vi "Read Scalar Data.vi"(8 "error in (no error)":errorcluster, 10 "Values":dbl[](array[numeric]), 11 "Cluster":T1 {"Data Type" format="%.0x"}) -> (0 "error out":errorcluster, 2 "Values":dbl[](array[numeric]), 3 "Cluster":T1 {"Data Type" format="%.0x"})   [LabVIEW 2019, in "FPGA Addon Engine.lvlib"]
uses:
  FPGA Addon Engine.lvlib
  Types/Register Settings.ctl
  Addon Shared/Types/Data Type.ctl
  Addon Shared/Types/Scalar Type.ctl
  <vilib>/Utility/error.llb/Error Cluster From Error Code.vi
  <vilib>/rvi/errors/niLvFpgaAdjustHostInterfaceError.vi
  <vilib>/rvi/interface/nirviReadWriteControl/nirviReadWriteControl.xnode
  NiFpgaLv.dll
  <vilib>/rvi/interface/Simulation/niFpgaSimulationCallBeginRW.vi
  Addon Shared/FPGA Addon Shared.lvlib
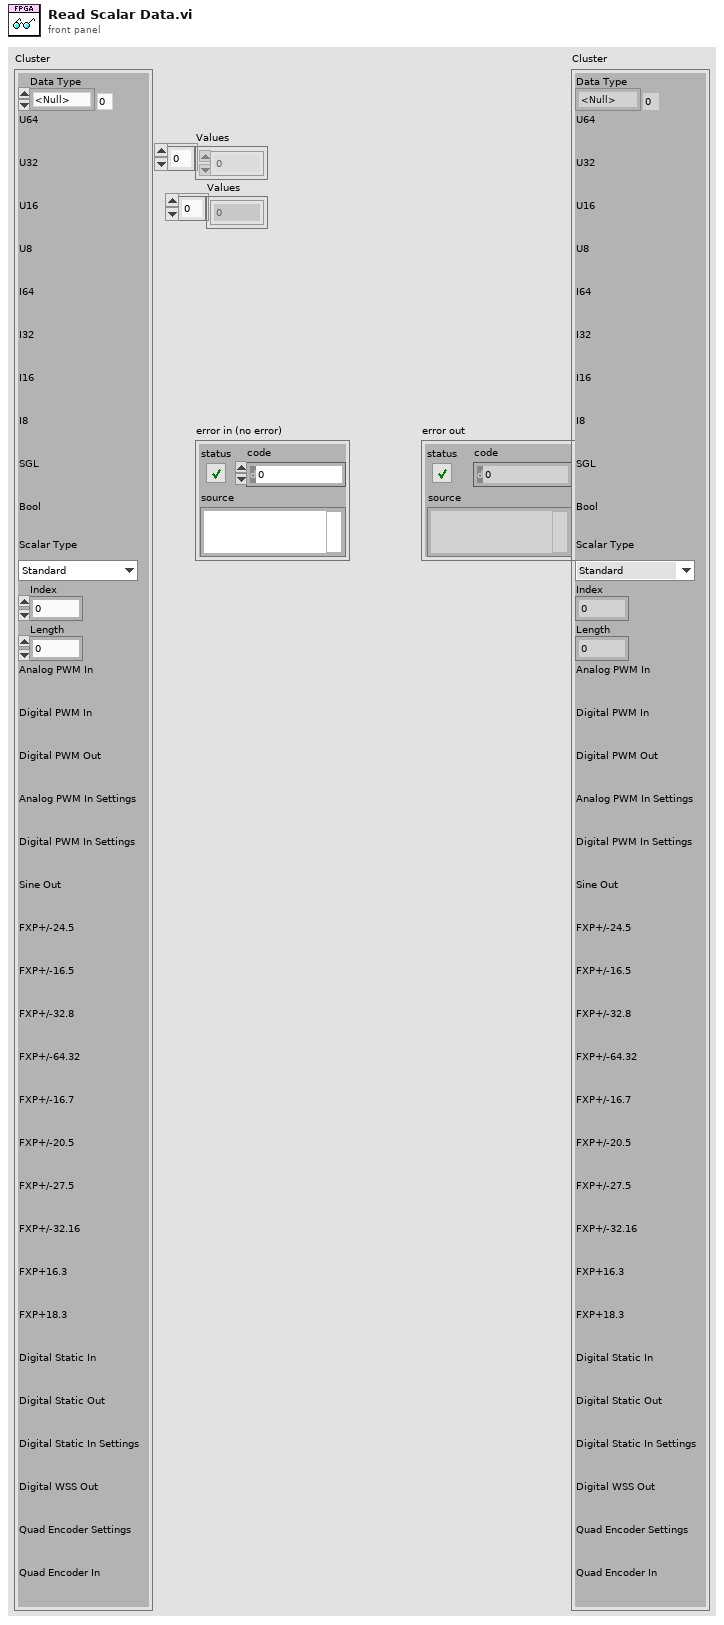
[diagram p1: front panel]
types:
  T1 = typedef "FPGA Addon Engine.lvlib/Register Settings.ctl" = cluster{"Data Type":T2, "U64":refnum<k20>, "U32":refnum<k20>, "U16":refnum<k20>, "U8":refnum<k20>, "I64":refnum<k20>, "I32":refnum<k20>, "I16":refnum<k20>, "I8":refnum<k20>, "SGL":refnum<k20>, "Bool":refnum<k20>, "Scalar Type":T3, "Index":i32, "Length":i32, "Analog PWM In":refnum<k20>, "Digital PWM In":refnum<k20>, "Digital PWM Out":refnum<k20>, "Analog PWM In Settings":refnum<k20>, "Digital PWM In Settings":refnum<k20>, "Sine Out":refnum<k20>, "FXP+/-24.5":refnum<k20>, "FXP+/-16.5":refnum<k20>, "FXP+/-32.8":refnum<k20>, "FXP+/-64.32":refnum<k20>, "FXP+/-16.7":refnum<k20>, "FXP+/-20.5":refnum<k20>, "FXP+/-27.5":refnum<k20>, "FXP+/-32.16":refnum<k20>, "FXP+16.3":refnum<k20>, "FXP+18.3":refnum<k20>, "Digital Static In":refnum<k20>, "Digital Static Out":refnum<k20>, "Digital Static In Settings":refnum<k20>, "Digital WSS Out":refnum<k20>, "Quad Encoder Settings":refnum<k20>, "Quad Encoder In":refnum<k20>}
  T2 = typedef "FPGA Addon Shared.lvlib/Data Type.ctl" = enum8{"<Null>", "I8", "I16", "I32", "I64", "U8", "U16", "U32", "U64", "SGL", "Boolean", "Analog PWM In Settings", "Analog PWM In", "Digital PWM In Settings", "Digital PWM In", "Digital PWM Out", "Sine Out", "FXP+/-24.5", "FXP+/-16.5", "FXP+/-32.8", "FXP+/-64.32", "FXP+/-16.7", "FXP+/-20.5", "FXP+/-27.5", "FXP+/-32.16", "FXP +16.3", "FXP +18.3", "Digital Static In", "Digital Static Out", "Digital Static In Settings", "Digital WSS Out", "Quad Encoder Settings", "Quad Encoder In"}
  T3 = typedef "FPGA Addon Shared.lvlib/Scalar Type.ctl" = enum16{"Standard", "Bitpacked"}
  T4 = cluster{"ACTIVE TICKS":u32, "INACTIVE TICKS":u32, "ACQ TICKS":u32, "ACTIVE VOLTAGE":fxp<+/-,32,8>, "INACTIVE VOLTAGE":fxp<+/-,32,8>}
  T5 = cluster{"ACTIVE TICKS":u32, "INACTIVE TICKS":u32, "ACQ TICKS":u32}
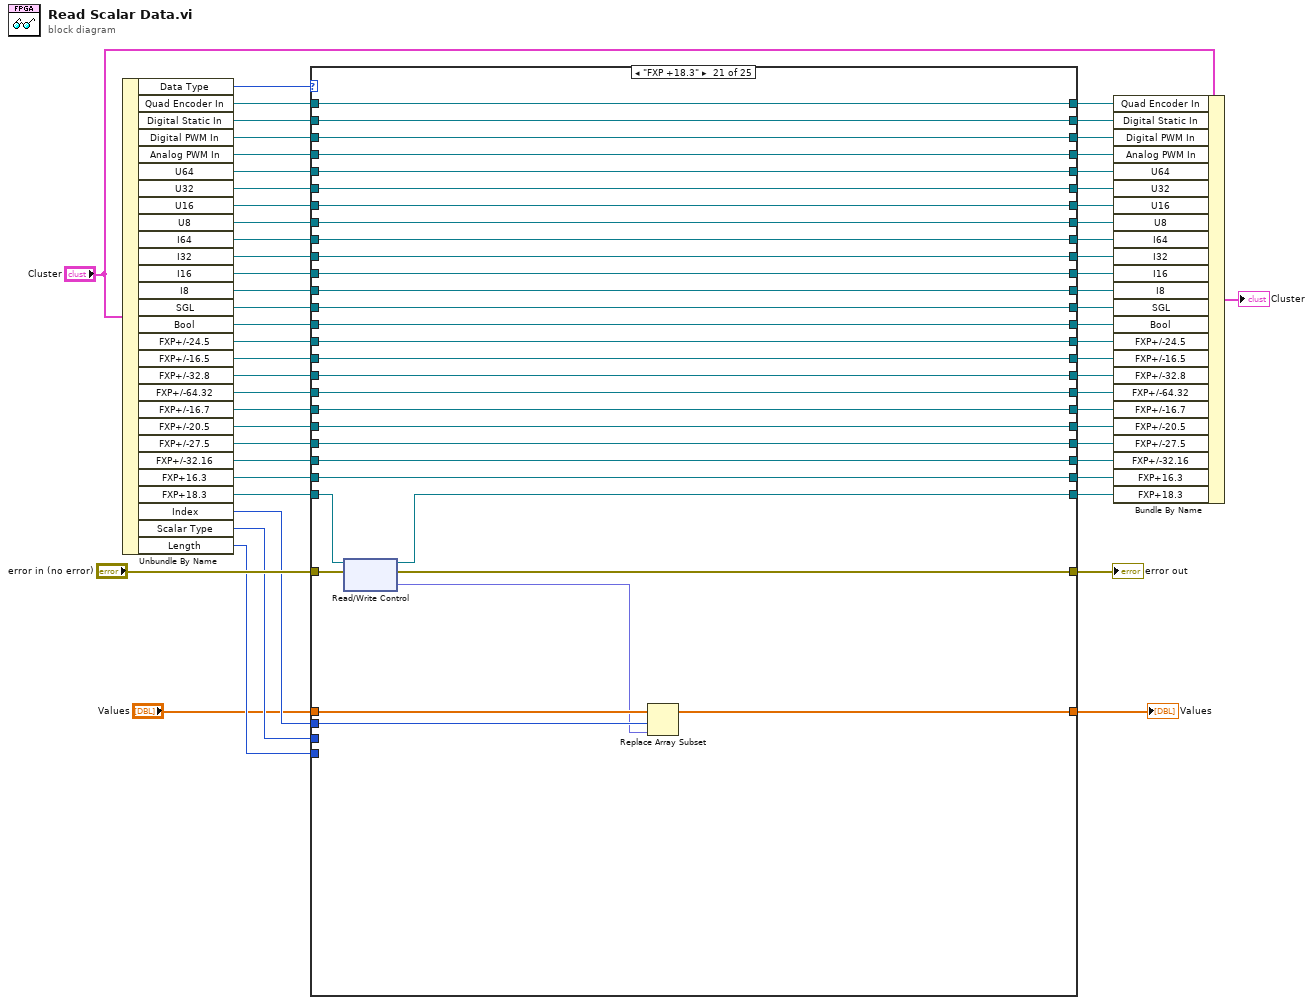
[diagram p0: block diagram]
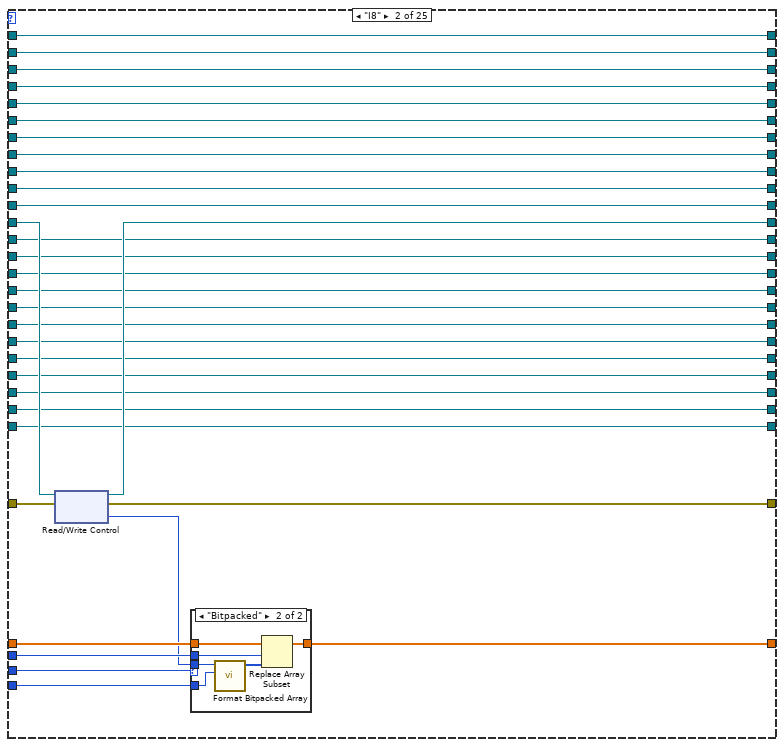
[diagram p3: hidden frame]
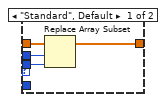
[diagram p4: hidden frame]
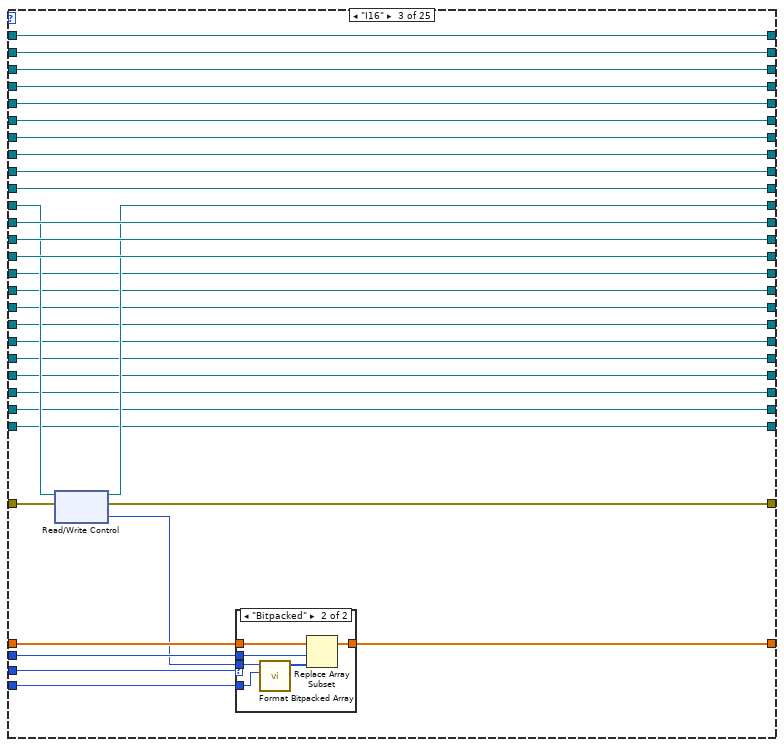
[diagram p5: hidden frame]
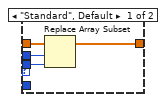
[diagram p6: hidden frame]
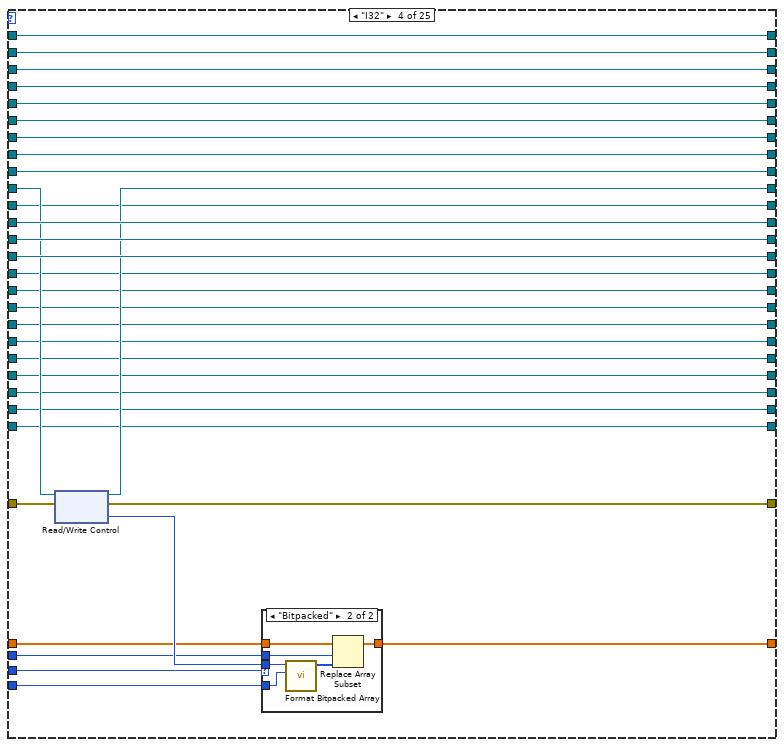
[diagram p7: hidden frame]
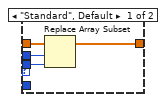
[diagram p8: hidden frame]
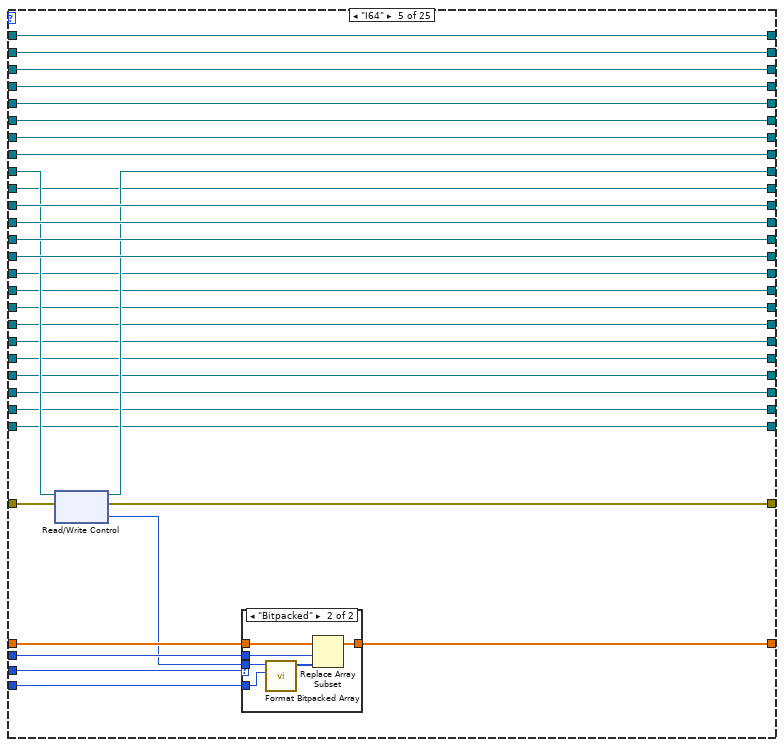
[diagram p9: hidden frame]
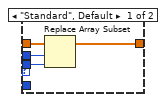
[diagram p10: hidden frame]
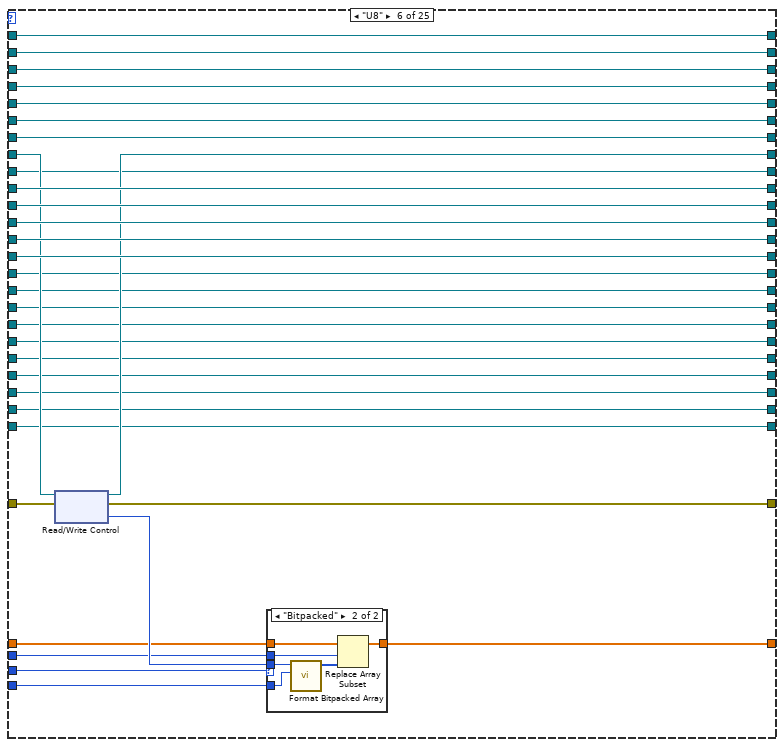
[diagram p11: hidden frame]
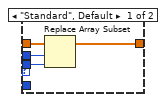
[diagram p12: hidden frame]
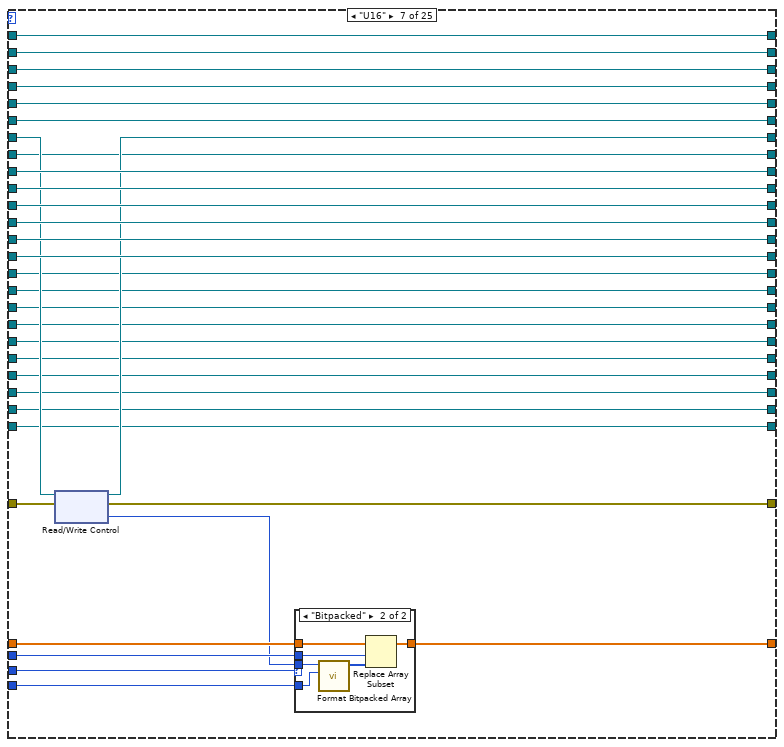
[diagram p13: hidden frame]
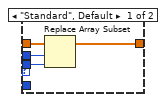
[diagram p14: hidden frame]
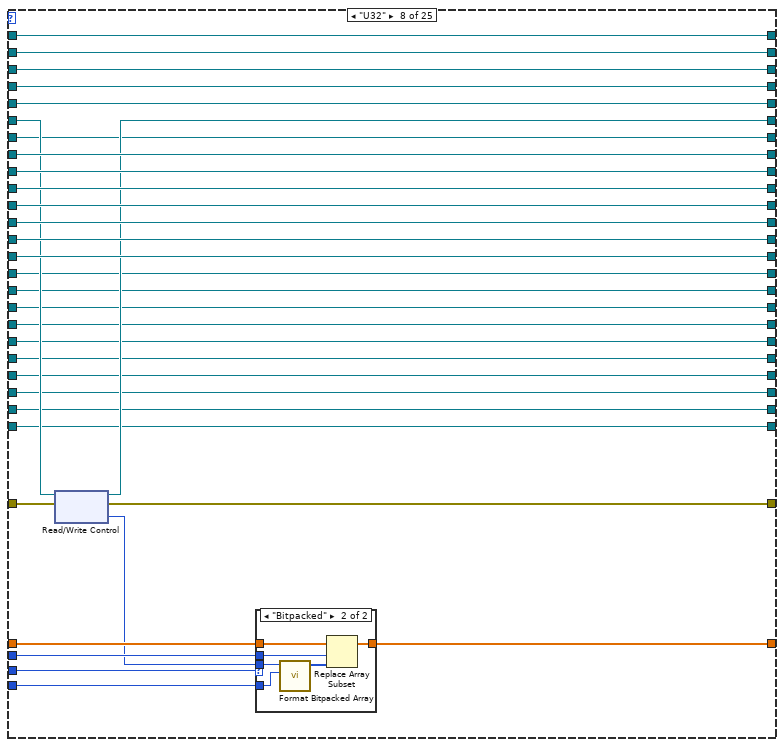
[diagram p15: hidden frame]
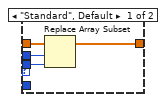
[diagram p16: hidden frame]
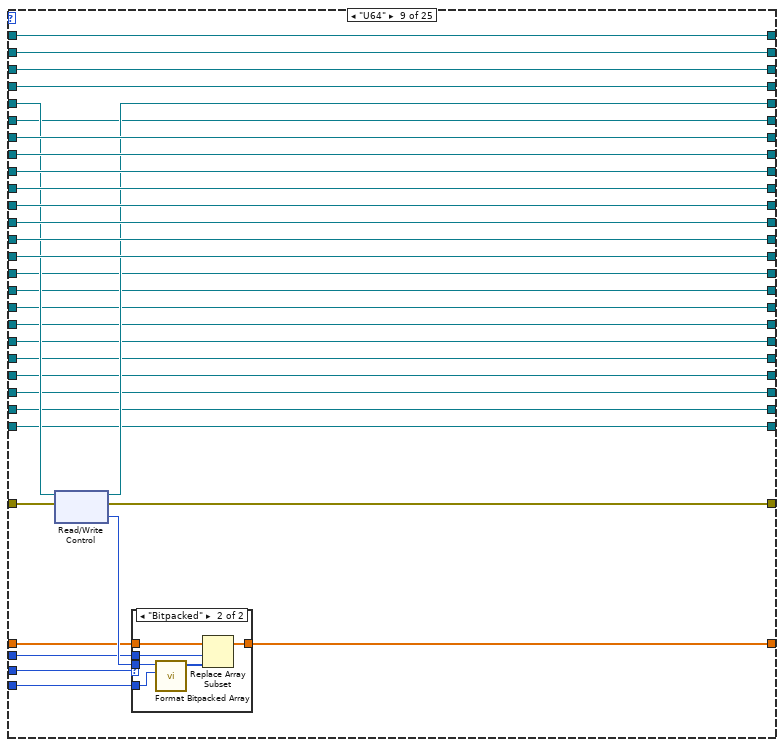
[diagram p17: hidden frame]
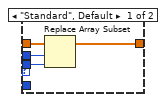
[diagram p18: hidden frame]
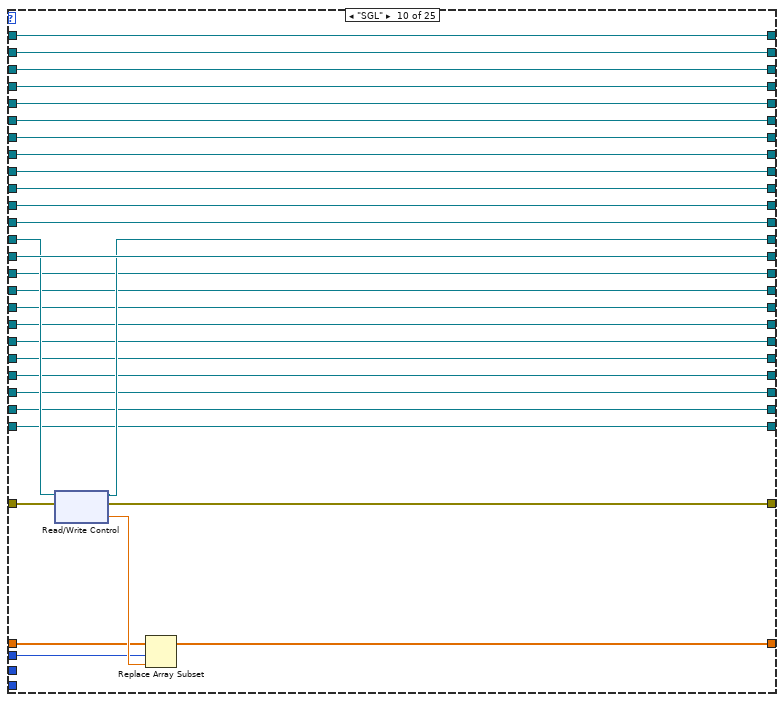
[diagram p19: hidden frame]
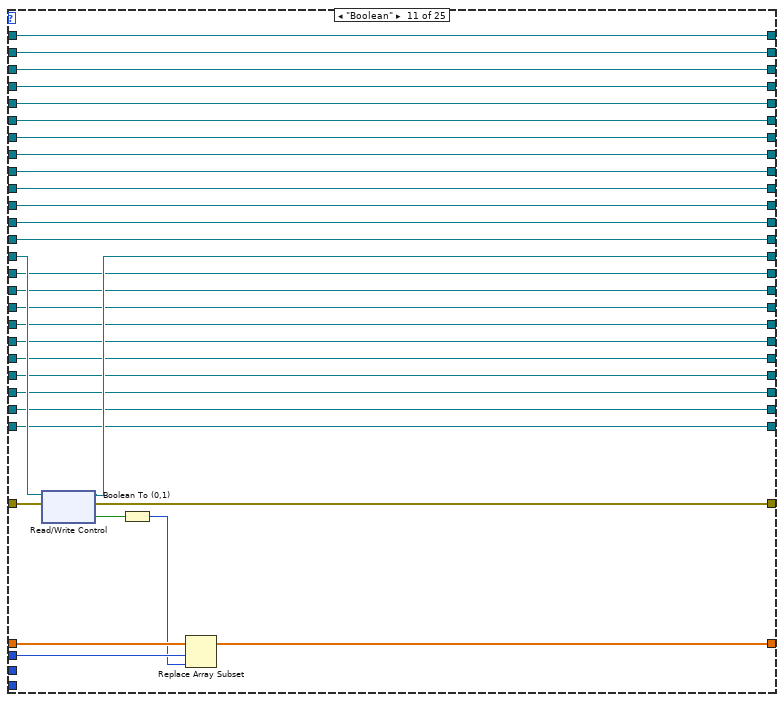
[diagram p20: hidden frame]
diagram:
  n1 = Unbundle By Name("Cluster") -> ("Data Type"=w7:T2, "Quad Encoder In"=w6:refnum<k20>, "Digital Static In"=w9:refnum<k20>, "Digital PWM In"=w27:refnum<k20>, "Analog PWM In"=w28:refnum<k20>, "U64"=w36:refnum<k20>, "U32"=w38:refnum<k20>, "U16"=w40:refnum<k20>, "U8"=w42:refnum<k20>, "I64"=w44:refnum<k20>, "I32"=w46:refnum<k20>, "I16"=w48:refnum<k20>, "I8"=w58:refnum<k20>, "SGL"=w52:refnum<k20>, "Bool"=w51:refnum<k20>, "FXP+/-24.5"=w25:refnum<k20>, "FXP+/-16.5"=w22:refnum<k20>, "FXP+/-32.8"=w21:refnum<k20>, "FXP+/-64.32"=w18:refnum<k20>, "FXP+/-16.7"=w16:refnum<k20>, "FXP+/-20.5"=w14:refnum<k20>, "FXP+/-27.5"=w13:refnum<k20>, "FXP+/-32.16"=w10:refnum<k20>, "FXP+16.3"=w3:refnum<k20>, "FXP+18.3"=w1:refnum<k20>, "Index"=w32:i32, "Scalar Type"=w33:T3, "Length"=w34:i32)
  n2 = case shown="\"FXP +18.3\"" w7 {
    tunnel: w58 -> [w82 w117 w150 w194 w238 w282 w326 w370 w414 w456 w489 w520 w551 w582 w613 w644 w675 w706 w737 w768 w799 w832 w878 w934 w971]
    tunnel: "error in (no error)" -> [w74 w116 w160 w203 w246 w289 w332 w375 w418 w459 w491 w522 w553 w584 w615 w646 w677 w708 w739 w770 w801 w834 w875 w931 w968]
    tunnel: [w74 w115 w159 w202 w245 w288 w331 w374 w417 w458 w490 w521 w552 w583 w614 w645 w676 w707 w738 w769 w800 w833 w874 w930 w967] -> w56
    tunnel: [w82 w114 w150 w194 w238 w282 w326 w370 w414 w456 w489 w520 w551 w582 w613 w644 w675 w706 w737 w768 w799 w832 w878 w934 w971] -> w54
    tunnel: [w83 w113 w158 w201 w244 w287 w330 w373 w416 w447 w479 w512 w543 w574 w605 w636 w667 w698 w729 w760 w791 w824 w877 w933 w970] -> w53
    tunnel: w52 -> [w83 w113 w158 w201 w244 w287 w330 w373 w416 w449 w479 w512 w543 w574 w605 w636 w667 w698 w729 w760 w791 w824 w877 w933 w970]
    tunnel: w51 -> [w84 w112 w157 w200 w243 w286 w329 w372 w415 w457 w481 w505 w537 w568 w599 w630 w661 w692 w723 w754 w785 w818 w876 w932 w969]
    tunnel: [w84 w112 w157 w200 w243 w286 w329 w372 w415 w457 w480 w505 w537 w568 w599 w630 w661 w692 w723 w754 w785 w818 w876 w932 w969] -> w50
    tunnel: [w81 w111 w148 w191 w237 w281 w325 w369 w413 w455 w488 w519 w550 w581 w612 w643 w674 w705 w736 w767 w798 w831 w879 w935 w972] -> w49
    tunnel: w48 -> [w81 w111 w149 w191 w237 w281 w325 w369 w413 w455 w488 w519 w550 w581 w612 w643 w674 w705 w736 w767 w798 w831 w879 w935 w972]
    tunnel: [w80 w110 w156 w192 w234 w280 w324 w368 w412 w454 w487 w518 w549 w580 w611 w642 w673 w704 w735 w766 w797 w830 w880 w936 w973] -> w47
    tunnel: w46 -> [w80 w110 w156 w193 w234 w280 w324 w368 w412 w454 w487 w518 w549 w580 w611 w642 w673 w704 w735 w766 w797 w830 w880 w936 w973]
    tunnel: [w79 w109 w155 w199 w235 w277 w323 w367 w411 w453 w486 w517 w548 w579 w610 w641 w672 w703 w734 w765 w796 w829 w881 w937 w974] -> w45
    tunnel: w44 -> [w79 w109 w155 w199 w236 w277 w323 w367 w411 w453 w486 w517 w548 w579 w610 w641 w672 w703 w734 w765 w796 w829 w881 w937 w974]
    tunnel: [w78 w108 w154 w198 w242 w278 w320 w366 w410 w452 w485 w516 w547 w578 w609 w640 w671 w702 w733 w764 w795 w828 w882 w938 w975] -> w43
    tunnel: w42 -> [w78 w108 w154 w198 w242 w279 w320 w366 w410 w452 w485 w516 w547 w578 w609 w640 w671 w702 w733 w764 w795 w828 w882 w938 w975]
    tunnel: [w77 w107 w153 w197 w241 w285 w321 w363 w409 w451 w484 w515 w546 w577 w608 w639 w670 w701 w732 w763 w794 w827 w883 w939 w976] -> w41
    tunnel: w40 -> [w77 w107 w153 w197 w241 w285 w322 w363 w409 w451 w484 w515 w546 w577 w608 w639 w670 w701 w732 w763 w794 w827 w883 w939 w976]
    tunnel: [w76 w106 w152 w196 w240 w284 w328 w364 w406 w450 w483 w514 w545 w576 w607 w638 w669 w700 w731 w762 w793 w826 w884 w940 w977] -> w39
    tunnel: w38 -> [w76 w106 w152 w196 w240 w284 w328 w365 w406 w450 w483 w514 w545 w576 w607 w638 w669 w700 w731 w762 w793 w826 w884 w940 w977]
    tunnel: [w75 w105 w151 w195 w239 w283 w327 w371 w407 w448 w482 w513 w544 w575 w606 w637 w668 w699 w730 w761 w792 w825 w885 w941 w978] -> w37
    tunnel: w36 -> [w75 w105 w151 w195 w239 w283 w327 w371 w408 w448 w482 w513 w544 w575 w606 w637 w668 w699 w730 w761 w792 w825 w885 w941 w978]
    tunnel: w34 -> [_ w101 w144 w185 w230 w273 w319 w358 w402 _ _ _ _ _ _ _ _ _ _ _ _ _ _ _ _]
    tunnel: w33 -> [_ w102 w145 w186 w231 w272 w318 w359 w403 _ _ _ _ _ _ _ _ _ _ _ _ _ _ _ _]
    tunnel: w32 -> [_ w103 w146 w189 w232 w274 w317 w360 w404 w445 w477 w511 w542 w573 w604 w635 w666 w697 w728 w759 w790 w823 w857 w913 w963]
    tunnel: "Values" -> [w73 w104 w147 w188 w233 w275 w316 w362 w401 w444 w476 w510 w541 w572 w603 w634 w665 w696 w727 w758 w789 w822 w859 w915 w965]
    tunnel: [w73 w99 w142 w187 w228 w271 w315 w361 w400 w443 w474 w509 w540 w571 w602 w633 w664 w695 w726 w757 w788 w821 w858 w914 w964] -> w30
    tunnel: [w72 w97 w140 w183 w226 w269 w312 w355 w398 w441 w472 w507 w538 w569 w600 w631 w662 w693 w724 w755 w786 w819 w872 w911 w962] -> w29
    tunnel: w28 -> [w72 w97 w140 w183 w226 w269 w312 w355 w398 w441 w472 w507 w538 w569 w600 w631 w662 w693 w724 w755 w786 w819 w873 w911 w962]
    tunnel: w27 -> [w71 w98 w141 w184 w227 w270 w313 w356 w399 w442 w473 w508 w539 w570 w601 w632 w663 w694 w725 w756 w787 w820 w886 w910 w952]
    tunnel: [w71 w98 w141 w184 w227 w270 w313 w356 w399 w442 w473 w508 w539 w570 w601 w632 w663 w694 w725 w756 w787 w820 w886 w909 w952] -> w26
    tunnel: w25 -> [w70 w96 w139 w182 w225 w268 w311 w354 w397 w440 w471 w506 w531 w565 w597 w628 w659 w690 w721 w752 w783 w816 w846 w903 w961]
    tunnel: [w70 w96 w139 w182 w225 w268 w311 w354 w397 w440 w471 w504 w531 w565 w597 w628 w659 w690 w721 w752 w783 w816 w846 w903 w961] -> w24
    tunnel: [w69 w95 w138 w181 w224 w267 w310 w353 w396 w439 w470 w502 w532 w564 w596 w627 w658 w689 w720 w751 w782 w815 w845 w902 w960] -> w23
    tunnel: w22 -> [w69 w95 w138 w181 w224 w267 w310 w353 w396 w439 w470 w502 w533 w564 w596 w627 w658 w689 w720 w751 w782 w815 w845 w902 w960]
    tunnel: w21 -> [w68 w94 w137 w180 w223 w266 w309 w352 w395 w438 w469 w501 w535 w563 w595 w626 w657 w688 w719 w750 w781 w814 w844 w901 w959]
    tunnel: [w68 w94 w137 w180 w223 w266 w309 w352 w395 w438 w469 w501 w535 w562 w595 w626 w657 w688 w719 w750 w781 w814 w844 w901 w959] -> w20
    tunnel: [w67 w93 w136 w179 w222 w265 w308 w351 w394 w437 w468 w500 w534 w566 w593 w625 w656 w687 w718 w749 w780 w813 w843 w900 w958] -> w19
    tunnel: w18 -> [w67 w93 w136 w179 w222 w265 w308 w351 w394 w437 w468 w500 w534 w566 w594 w625 w656 w687 w718 w749 w780 w813 w843 w900 w958]
    tunnel: [w66 w92 w135 w178 w221 w264 w307 w350 w393 w436 w467 w499 w530 w561 w592 w623 w653 w686 w717 w748 w779 w812 w842 w899 w957] -> w17
    tunnel: w16 -> [w66 w92 w135 w178 w221 w264 w307 w350 w393 w436 w467 w499 w530 w561 w592 w624 w653 w686 w717 w748 w779 w812 w842 w899 w957]
    tunnel: [w65 w91 w134 w177 w220 w263 w306 w349 w392 w435 w466 w498 w529 w560 w591 w622 w655 w684 w716 w747 w778 w811 w841 w898 w956] -> w15
    tunnel: w14 -> [w65 w91 w134 w177 w220 w263 w306 w349 w392 w435 w466 w498 w529 w560 w591 w622 w654 w684 w716 w747 w778 w811 w841 w898 w956]
    tunnel: w13 -> [w64 w90 w133 w176 w219 w262 w305 w348 w391 w434 w465 w497 w528 w559 w590 w621 w652 w685 w715 w746 w777 w810 w840 w897 w955]
    tunnel: [w64 w90 w133 w176 w219 w262 w305 w348 w391 w434 w465 w497 w528 w559 w590 w621 w652 w683 w715 w746 w777 w810 w840 w897 w955] -> w12
    tunnel: [w63 w89 w132 w175 w218 w261 w304 w347 w390 w433 w464 w496 w527 w558 w589 w620 w651 w682 w713 w742 w774 w805 w839 w896 w954] -> w11
    tunnel: w10 -> [w63 w89 w132 w175 w218 w261 w304 w347 w390 w433 w464 w496 w527 w558 w589 w620 w651 w682 w714 w742 w774 w805 w839 w896 w954]
    tunnel: w9 -> [w62 w88 w131 w174 w217 w260 w303 w346 w389 w432 w463 w495 w526 w557 w588 w619 w650 w681 w712 w745 w776 w809 w838 w895 w953]
    tunnel: [w62 w88 w131 w174 w217 w260 w303 w346 w389 w432 w463 w495 w526 w557 w588 w619 w650 w681 w712 w745 w776 w807 w838 w895 w953] -> w8
    tunnel: w6 -> [w61 w87 w130 w173 w216 w259 w302 w345 w388 w431 w462 w494 w525 w556 w587 w618 w649 w680 w711 w744 w775 w804 w837 w894 w951]
    tunnel: [w61 w87 w130 w173 w216 w259 w302 w345 w388 w431 w462 w494 w525 w556 w587 w618 w649 w680 w711 w744 w775 w804 w837 w894 w950] -> w5
    tunnel: [w59 w85 w128 w171 w214 w257 w300 w343 w386 w429 w460 w492 w523 w554 w585 w616 w647 w678 w710 w740 w773 w802 w835 w892 w947] -> w4
    tunnel: w3 -> [w59 w85 w128 w171 w214 w257 w300 w343 w386 w429 w460 w492 w523 w554 w585 w616 w647 w678 w710 w741 w773 w802 w835 w892 w947]
    tunnel: [w60 w86 w129 w172 w215 w258 w301 w344 w387 w430 w461 w493 w524 w555 w586 w617 w648 w679 w709 w743 w771 w803 w836 w893 w948] -> w2
    tunnel: w1 -> [w60 w86 w129 w172 w215 w258 w301 w344 w387 w430 w461 w493 w524 w555 w586 w617 w648 w679 w709 w743 w772 w803 w836 w893 w948]
    frame "<Null>", Default {
    }
    frame "I8" {
      n3 = xnode "Read/Write Control"("FPGA VI Reference In"=w117, "error in"=w116) -> ("FPGA VI Reference Out"=w114:refnum<k20>, "error out"=w115:errorcluster, "Value"=w100:i8)
      n4 = case shown="\"Bitpacked\"" w102 {
        tunnel: w104 -> [w121 w125]
        tunnel: [w120 w124] -> w99
        tunnel: w100 -> [w119 w127]
        tunnel: w103 -> [w118 w122]
        tunnel: w101 -> [_ w126]
        frame "Standard", Default {
          n5 = Replace Array Subset(array=w121, new element=w119, index=w118) -> (w120:dbl[])
        }
        frame "Bitpacked" {
          n6 = call "Format Bitpacked Array.vi"("Length"=w126, "Value"=w127) -> ("Array"=w123:i16[])  [unwired: 9 in]
          n7 = Replace Array Subset(array=w125, new element=w123, index=w122) -> (w124:dbl[])
        }
      }
    }
    frame "I16" {
      n8 = xnode "Read/Write Control"("FPGA VI Reference In"=w149, "error in"=w160) -> ("FPGA VI Reference Out"=w148:refnum<k20>, "error out"=w159:errorcluster, "Value"=w143:i16)
      n9 = case shown="\"Bitpacked\"" w145 {
        tunnel: w147 -> [w164 w168]
        tunnel: [w163 w167] -> w142
        tunnel: w143 -> [w162 w170]
        tunnel: w146 -> [w161 w165]
        tunnel: w144 -> [_ w169]
        frame "Standard", Default {
          n10 = Replace Array Subset(array=w164, new element=w162, index=w161) -> (w163:dbl[])
        }
        frame "Bitpacked" {
          n11 = call "Format Bitpacked Array.vi"("Length"=w169, "Value"=w170) -> ("Array"=w166:i16[])  [unwired: 9 in]
          n12 = Replace Array Subset(array=w168, new element=w166, index=w165) -> (w167:dbl[])
        }
      }
    }
    frame "I32" {
      n13 = xnode "Read/Write Control"("FPGA VI Reference In"=w193, "error in"=w203) -> ("FPGA VI Reference Out"=w192:refnum<k20>, "error out"=w202:errorcluster, "Value"=w190:i32)
      n14 = case shown="\"Bitpacked\"" w186 {
        tunnel: w188 -> [w207 w211]
        tunnel: [w206 w210] -> w187
        tunnel: w190 -> [w205 w213]
        tunnel: w189 -> [w204 w208]
        tunnel: w185 -> [_ w212]
        frame "Standard", Default {
          n15 = Replace Array Subset(array=w207, new element=w205, index=w204) -> (w206:dbl[])
        }
        frame "Bitpacked" {
          n16 = call "Format Bitpacked Array.vi"("Length"=w212, "Value"=w213) -> ("Array"=w209:i16[])  [unwired: 9 in]
          n17 = Replace Array Subset(array=w211, new element=w209, index=w208) -> (w210:dbl[])
        }
      }
    }
    frame "I64" {
      n18 = xnode "Read/Write Control"("FPGA VI Reference In"=w236, "error in"=w246) -> ("FPGA VI Reference Out"=w235:refnum<k20>, "error out"=w245:errorcluster, "Value"=w229:i64)
      n19 = case shown="\"Bitpacked\"" w231 {
        tunnel: w233 -> [w250 w254]
        tunnel: [w249 w253] -> w228
        tunnel: w229 -> [w248 w256]
        tunnel: w232 -> [w247 w251]
        tunnel: w230 -> [_ w255]
        frame "Standard", Default {
          n20 = Replace Array Subset(array=w250, new element=w248, index=w247) -> (w249:dbl[])
        }
        frame "Bitpacked" {
          n21 = call "Format Bitpacked Array.vi"("Length"=w255, "Value"=w256) -> ("Array"=w252:i16[])  [unwired: 9 in]
          n22 = Replace Array Subset(array=w254, new element=w252, index=w251) -> (w253:dbl[])
        }
      }
    }
    frame "U8" {
      n23 = xnode "Read/Write Control"("FPGA VI Reference In"=w279, "error in"=w289) -> ("FPGA VI Reference Out"=w278:refnum<k20>, "error out"=w288:errorcluster, "Value"=w276:u8)
      n24 = case shown="\"Bitpacked\"" w272 {
        tunnel: w275 -> [w293 w297]
        tunnel: [w292 w296] -> w271
        tunnel: w276 -> [w291 w299]
        tunnel: w274 -> [w290 w294]
        tunnel: w273 -> [_ w298]
        frame "Standard", Default {
          n25 = Replace Array Subset(array=w293, new element=w291, index=w290) -> (w292:dbl[])
        }
        frame "Bitpacked" {
          n26 = call "Format Bitpacked Array.vi"("Length"=w298, "Value"=w299) -> ("Array"=w295:i16[])  [unwired: 9 in]
          n27 = Replace Array Subset(array=w297, new element=w295, index=w294) -> (w296:dbl[])
        }
      }
    }
    frame "U16" {
      n28 = xnode "Read/Write Control"("FPGA VI Reference In"=w322, "error in"=w332) -> ("FPGA VI Reference Out"=w321:refnum<k20>, "error out"=w331:errorcluster, "Value"=w314:u16)
      n29 = case shown="\"Bitpacked\"" w318 {
        tunnel: w316 -> [w336 w340]
        tunnel: [w335 w339] -> w315
        tunnel: w314 -> [w334 w342]
        tunnel: w317 -> [w333 w337]
        tunnel: w319 -> [_ w341]
        frame "Standard", Default {
          n30 = Replace Array Subset(array=w336, new element=w334, index=w333) -> (w335:dbl[])
        }
        frame "Bitpacked" {
          n31 = call "Format Bitpacked Array.vi"("Length"=w341, "Value"=w342) -> ("Array"=w338:i16[])  [unwired: 9 in]
          n32 = Replace Array Subset(array=w340, new element=w338, index=w337) -> (w339:dbl[])
        }
      }
    }
    frame "U32" {
      n33 = xnode "Read/Write Control"("FPGA VI Reference In"=w365, "error in"=w375) -> ("FPGA VI Reference Out"=w364:refnum<k20>, "error out"=w374:errorcluster, "Value"=w357:u32)
      n34 = case shown="\"Bitpacked\"" w359 {
        tunnel: w362 -> [w379 w383]
        tunnel: [w378 w382] -> w361
        tunnel: w357 -> [w377 w385]
        tunnel: w360 -> [w376 w380]
        tunnel: w358 -> [_ w384]
        frame "Standard", Default {
          n35 = Replace Array Subset(array=w379, new element=w377, index=w376) -> (w378:dbl[])
        }
        frame "Bitpacked" {
          n36 = call "Format Bitpacked Array.vi"("Length"=w384, "Value"=w385) -> ("Array"=w381:i16[])  [unwired: 9 in]
          n37 = Replace Array Subset(array=w383, new element=w381, index=w380) -> (w382:dbl[])
        }
      }
    }
    frame "U64" {
      n38 = xnode "Read/Write Control"("FPGA VI Reference In"=w408, "error in"=w418) -> ("FPGA VI Reference Out"=w407:refnum<k20>, "error out"=w417:errorcluster, "Value"=w405:u64)
      n39 = case shown="\"Bitpacked\"" w403 {
        tunnel: w401 -> [w422 w426]
        tunnel: [w421 w425] -> w400
        tunnel: w405 -> [w420 w428]
        tunnel: w404 -> [w419 w423]
        tunnel: w402 -> [_ w427]
        frame "Standard", Default {
          n40 = Replace Array Subset(array=w422, new element=w420, index=w419) -> (w421:dbl[])
        }
        frame "Bitpacked" {
          n41 = call "Format Bitpacked Array.vi"("Length"=w427, "Value"=w428) -> ("Array"=w424:i16[])  [unwired: 9 in]
          n42 = Replace Array Subset(array=w426, new element=w424, index=w423) -> (w425:dbl[])
        }
      }
    }
    frame "SGL" {
      n43 = xnode "Read/Write Control"("FPGA VI Reference In"=w449, "error in"=w459) -> ("FPGA VI Reference Out"=w447:refnum<k20>, "error out"=w458:errorcluster, "Value"=w446:sgl)
      n44 = Replace Array Subset(array=w444, new element=w446, index=w445) -> (w443:dbl[])
    }
    frame "Boolean" {
      n45 = xnode "Read/Write Control"("FPGA VI Reference In"=w481, "error in"=w491) -> ("FPGA VI Reference Out"=w480:refnum<k20>, "error out"=w490:errorcluster, "Value"=w478:bool)
      n46 = Boolean To (0,1)(Boolean=w478) -> (0, 1=w475:i16)
      n47 = Replace Array Subset(array=w476, new element=w475, index=w477) -> (w474:dbl[])
    }
    frame "FXP+/-24.5" {
      n48 = xnode "Read/Write Control"("FPGA VI Reference In"=w506, "error in"=w522) -> ("FPGA VI Reference Out"=w504:refnum<k20>, "error out"=w521:errorcluster, "Value"=w503:fxp<+/-,24,5>)
      n49 = Replace Array Subset(array=w510, new element=w503, index=w511) -> (w509:dbl[])
    }
    frame "FXP+/-16.5" {
      n50 = xnode "Read/Write Control"("FPGA VI Reference In"=w533, "error in"=w553) -> ("FPGA VI Reference Out"=w532:refnum<k20>, "error out"=w552:errorcluster, "Value"=w536:fxp<+/-,16,5>)
      n51 = Replace Array Subset(array=w541, new element=w536, index=w542) -> (w540:dbl[])
    }
    frame "FXP+/-32.8" {
      n52 = xnode "Read/Write Control"("FPGA VI Reference In"=w563, "error in"=w584) -> ("FPGA VI Reference Out"=w562:refnum<k20>, "error out"=w583:errorcluster, "Value"=w567:fxp<+/-,32,8>)
      n53 = Replace Array Subset(array=w572, new element=w567, index=w573) -> (w571:dbl[])
    }
    frame "FXP+/-64.32" {
      n54 = xnode "Read/Write Control"("FPGA VI Reference In"=w594, "error in"=w615) -> ("FPGA VI Reference Out"=w593:refnum<k20>, "error out"=w614:errorcluster, "Value"=w598:fxp<+/-,64,32>)
      n55 = Replace Array Subset(array=w603, new element=w598, index=w604) -> (w602:dbl[])
    }
    frame "FXP+/-16.7" {
      n56 = xnode "Read/Write Control"("FPGA VI Reference In"=w624, "error in"=w646) -> ("FPGA VI Reference Out"=w623:refnum<k20>, "error out"=w645:errorcluster, "Value"=w629:fxp<+/-,16,7>)
      n57 = Replace Array Subset(array=w634, new element=w629, index=w635) -> (w633:dbl[])
    }
    frame "FXP+/-20.5" {
      n58 = xnode "Read/Write Control"("FPGA VI Reference In"=w654, "error in"=w677) -> ("FPGA VI Reference Out"=w655:refnum<k20>, "error out"=w676:errorcluster, "Value"=w660:fxp<+/-,20,5>)
      n59 = Replace Array Subset(array=w665, new element=w660, index=w666) -> (w664:dbl[])
    }
    frame "FXP+/-27.5" {
      n60 = xnode "Read/Write Control"("FPGA VI Reference In"=w685, "error in"=w708) -> ("FPGA VI Reference Out"=w683:refnum<k20>, "error out"=w707:errorcluster, "Value"=w691:fxp<+/-,27,5>)
      n61 = Replace Array Subset(array=w696, new element=w691, index=w697) -> (w695:dbl[])
    }
    frame "FXP+/-32.16" {
      n62 = xnode "Read/Write Control"("FPGA VI Reference In"=w714, "error in"=w739) -> ("FPGA VI Reference Out"=w713:refnum<k20>, "error out"=w738:errorcluster, "Value"=w722:fxp<+/-,32,16>)
      n63 = Replace Array Subset(array=w727, new element=w722, index=w728) -> (w726:dbl[])
    }
    frame "FXP +16.3" {
      n64 = xnode "Read/Write Control"("FPGA VI Reference In"=w741, "error in"=w770) -> ("FPGA VI Reference Out"=w740:refnum<k20>, "error out"=w769:errorcluster, "Value"=w753:fxp<+,16,3>)
      n65 = Replace Array Subset(array=w758, new element=w753, index=w759) -> (w757:dbl[])
    }
    frame "FXP +18.3" {
      n66 = xnode "Read/Write Control"("FPGA VI Reference In"=w772, "error in"=w801) -> ("FPGA VI Reference Out"=w771:refnum<k20>, "error out"=w800:errorcluster, "Value"=w784:fxp<+,18,3>)
      n67 = Replace Array Subset(array=w789, new element=w784, index=w790) -> (w788:dbl[])
    }
    frame "Digital Static In" {
      n68 = xnode "Read/Write Control"("FPGA VI Reference In"=w809, "error in"=w834) -> ("FPGA VI Reference Out"=w807:refnum<k20>, "error out"=w833:errorcluster, "Value"=w817:cluster{"STATE":bool})
      n69 = Unbundle By Name(w817) -> ("STATE"=w808:bool)
      n70 = Boolean To (0,1)(Boolean=w808) -> (0, 1=w806:i16)
      n71 = Replace Array Subset(array=w822, new element=w806, index=w823) -> (w821:dbl[])
    }
    frame "Analog PWM In" {
      w866 = 2.5000000292152436e-08 ("y")
      n72 = xnode "Read/Write Control"("FPGA VI Reference In"=w873, "error in"=w875) -> ("FPGA VI Reference Out"=w872:refnum<k20>, "error out"=w874:errorcluster, "Value"=w854:T4)
      n73 = Unbundle By Name(w854) -> ("ACTIVE TICKS"=w853:u32, "INACTIVE TICKS"=w852:u32, "ACQ TICKS"=w851:u32, "ACTIVE VOLTAGE"=w850:fxp<+/-,32,8>, "INACTIVE VOLTAGE"=w849:fxp<+/-,32,8>)
      n74 = Add(x=w853, y=w852) -> (x+y=w868:u32)
      n75 = Compound Arithmetic op=MULTIPLY(w868, w851, w866) -> (w869:dbl)
      n76 = Divide(x=w853, y=w868) -> (x/y=w862:dbl)
      n77 = Compound Arithmetic op=MULTIPLY(w853, w851, w866) -> (w867:dbl)
      n78 = Multiply(x=100.0, y=w862) -> (x*y=w861:dbl)
      n79 = Equal?(x=0.0, y=w869) -> (x = y?=w865:bool)
      n80 = Reciprocal(x=w869) -> (1/x=w870:dbl)
      n81 = case shown="False" w865 {
        tunnel: [w887 w891] -> w848
        tunnel: [w888 w891] -> w855
        tunnel: [w890 w891] -> w847
        tunnel: w869 -> [w890 _]
        tunnel: [w889 w891] -> w860
        tunnel: w867 -> [w889 _]
        tunnel: w861 -> [w888 _]
        tunnel: w870 -> [w887 _]
        tunnel: 0.0 ("x") -> [_ w891]
        frame False {
        }
        frame True {
        }
      }
      n82 = Build Array(w848, w847, w855, w860, w850, w849) -> (w856:dbl[])
      n83 = Replace Array Subset(array=w859, new element=w856, index=w857) -> (w858:dbl[])
    }
    frame "Digital PWM In" {
      w924 = 2.5000000292152436e-08 ("y")
      n84 = xnode "Read/Write Control"("FPGA VI Reference In"=w910, "error in"=w931) -> ("FPGA VI Reference Out"=w909:refnum<k20>, "error out"=w930:errorcluster, "Value"=w917:T5)
      n85 = Unbundle By Name(w917) -> ("ACTIVE TICKS"=w907:u32, "INACTIVE TICKS"=w906:u32, "ACQ TICKS"=w920:u32)
      n86 = Add(x=w907, y=w906) -> (x+y=w926:u32)
      n87 = Compound Arithmetic op=MULTIPLY(w926, w920, w924) -> (w927:dbl)
      n88 = Divide(x=w907, y=w926) -> (x/y=w919:dbl)
      n89 = Compound Arithmetic op=MULTIPLY(w907, w920, w924) -> (w925:dbl)
      n90 = Multiply(x=100.0, y=w919) -> (x*y=w918:dbl)
      n91 = Equal?(x=0.0, y=w927) -> (x = y?=w923:bool)
      n92 = Reciprocal(x=w927) -> (1/x=w928:dbl)
      n93 = case shown="False" w923 {
        tunnel: [w942 w946] -> w905
        tunnel: [w943 w946] -> w908
        tunnel: [w945 w946] -> w904
        tunnel: w927 -> [w945 _]
        tunnel: [w944 w946] -> w916
        tunnel: w925 -> [w944 _]
        tunnel: w918 -> [w943 _]
        tunnel: w928 -> [w942 _]
        tunnel: 0.0 ("x") -> [_ w946]
        frame False {
        }
        frame True {
        }
      }
      n94 = Build Array(w905, w904, w908, w916) -> (w912:dbl[])
      n95 = Replace Array Subset(array=w915, new element=w912, index=w913) -> (w914:dbl[])
    }
    frame "Quad Encoder In" {
      n96 = xnode "Read/Write Control"("FPGA VI Reference In"=w951, "error in"=w968) -> ("FPGA VI Reference Out"=w950:refnum<k20>, "error out"=w967:errorcluster, "Value"=w966:cluster{"POSITION":i32})
      n97 = Unbundle By Name(w966) -> ("POSITION"=w949:i32)
      n98 = Replace Array Subset(array=w965, new element=w949, index=w963) -> (w964:dbl[])
    }
  }
  "error out" <- w56
  "Values" <- w30
  n99 = Bundle By Name(cluster="Cluster", "Quad Encoder In"=w5, "Digital Static In"=w8, "Digital PWM In"=w26, "Analog PWM In"=w29, "U64"=w37, "U32"=w39, "U16"=w41, "U8"=w43, "I64"=w45, "I32"=w47, "I16"=w49, "I8"=w54, "SGL"=w53, "Bool"=w50, "FXP+/-24.5"=w24, "FXP+/-16.5"=w23, "FXP+/-32.8"=w20, "FXP+/-64.32"=w19, "FXP+/-16.7"=w17, "FXP+/-20.5"=w15, "FXP+/-27.5"=w12, "FXP+/-32.16"=w11, "FXP+16.3"=w4, "FXP+18.3"=w2) -> (→"Cluster":T1)
